vi "GenerateEventUpdateList.vi"(9 "ProjectItem":refnum<class "ProjectItem.lvclass">, 11 "UpdateList":T1) -> ()   [LabVIEW 2019, in "SolutionBuilder.lvlib" / "ProjectItem.lvclass"]
uses:
  ProjectItem.lvclass
  Events/EventUpdateList.ctl
  ProjectItem.lvclass/ProjectItem.ctl
  SolutionBuilder.lvlib
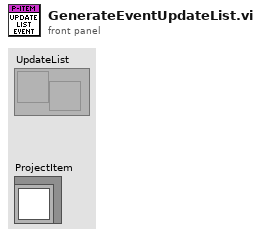
[diagram p1: front panel]
types:
  T1 = typedef "SolutionBuilder.lvlib/EventUpdateList.ctl" = refnum<user-event>
  T2 = cluster{"Build spec name":string, "Target":string, "Owning lib name":string, "name":string}
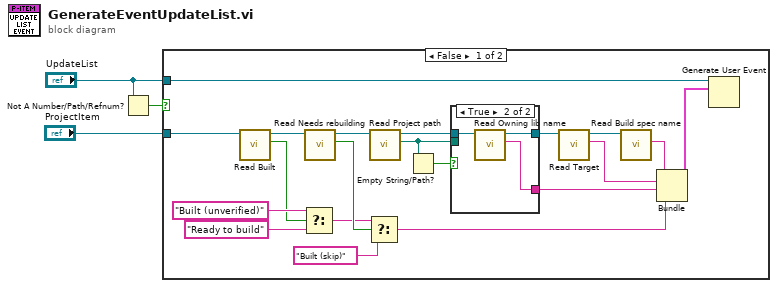
[diagram p0: block diagram]
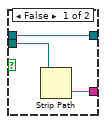
[diagram p2: hidden frame]
diagram:
  n1 = Not A Number/Path/Refnum?(number/path/refnum="UpdateList") -> (NaN/Path/Refnum?=w1:bool)
  n2 = case shown="False" w1 {
    tunnel: "ProjectItem" -> [w23 _]
    tunnel: "UpdateList" -> [w18 _]
    frame False {
      n3 = call-dynamic "Read Built.vi"("ProjectItem in"=w23) -> ("Built"=w15:bool, "ProjectItem out"=w9:refnum<class "ProjectItem.lvclass">)  [unwired: 9 in]
      n4 = Select(t="Built (unverified)" ("name"), s=w15, f="Ready to build" ("name")) -> (s? t:f=w6:string)
      n5 = call-dynamic "Read Needs rebuilding.vi"("ProjectItem in"=w9) -> ("Needs rebuilding"=w7:bool, "ProjectItem out"=w8:refnum<class "ProjectItem.lvclass">)  [unwired: 9 in]
      n6 = Select(t=w6, s=w7, f="Built (skip)" ("name")) -> (s? t:f=w5:string)
      n7 = call-dynamic "Read Project path.vi"("ProjectItem in"=w8) -> ("Project path"=w13:path, "ProjectItem out"=w14:refnum<class "ProjectItem.lvclass">)  [unwired: 9 in]
      n8 = Empty String/Path?(string/path=w13) -> (empty?=w12:bool)
      n9 = case shown="True" w12 {
        tunnel: w14 -> [w25 w29]
        tunnel: [w26 w27] -> w11
        tunnel: [w25 w28] -> w10
        tunnel: w13 -> [w24 _]
        frame False {
          n10 = Strip Path(path=w24) -> (name=w26:string)  [unwired: 1 out]
        }
        frame True {
          n11 = call-dynamic "Read Owning lib name.vi"("ProjectItem in"=w29) -> ("Owning lib name"=w27:string, "ProjectItem out"=w28:refnum<class "ProjectItem.lvclass">)  [unwired: 9 in]
        }
      }
      n12 = call "Read Target.vi"("ProjectItem in"=w10) -> ("Target"=w16:string, "ProjectItem out"=w17:refnum<class "ProjectItem.lvclass">)  [unwired: 9 in]
      n13 = call-dynamic "Read Build spec name.vi"("ProjectItem in"=w17) -> ("Build spec name"=w22:string)  [unwired: 9 in, 1 out]
      n14 = Bundle("Build spec name"=w22, "Target"=w16, "Owning lib name"=w11, "name"=w5) -> (w19:T2)  [unwired: 1 in]
      n15 = Generate User Event(user event=w18, event data cluster=w19) -> ()  [unwired: 2 in, 2 out]
    }
    frame True {
    }
  }
